vi "create event from asset.vi"(7 "Time Stamp (now)":timestamp format="%<%x %.3X>T", 9 "Type":enum16{"INFO", "FLAG", "ERROR", "SUCCESS"}(ring), 10 "Name":string, 11 "asset":refnum<class "asset.lvclass">) -> (0 "error out":errorcluster, 3 "event":refnum<class "event.lvclass">)   [LabVIEW 2020, in "nominal core steps.lvlib"]
doc: "Creates a named event associated with a specific asset."
uses:
  nominal core steps.lvlib
  <vilib>/Nominal/Nominal IO Client/lv_src/event/event.lvclass
  <vilib>/Nominal/Nominal IO Client/lv_src/asset/asset.lvclass
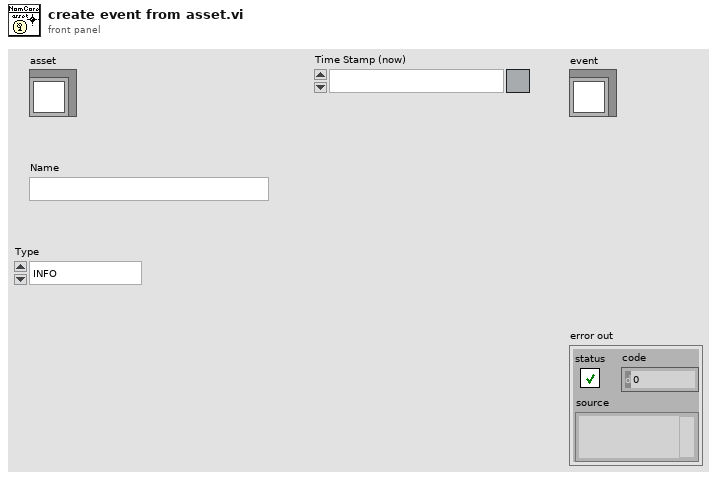
[diagram p1: front panel]
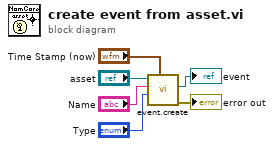
[diagram p0: block diagram]
diagram:
  n1 = call <vilib>:"event.create.vi"("Time Stamp (now)"="Time Stamp (now)", "Type"="Type", "Name"="Name", "asset in"="asset") -> ("error out"=→"error out":errorcluster, "event"=→"event":refnum<class "event.lvclass">)  [unwired: 5 in, 1 out]
